vi "Process Records.vi"(4 "map from message info to indexes":T2, 5 "RT hardware channel data":T3[](array[typedef])=[{"channel #"=0, "channel handle"=0, "labels settings for RT"=[]}] {"labels settings for RT"."Label Timestamp Channel Data Reference" format="%.0x"; "labels settings for RT"."Word Initial Raw Value" format="%032.0f"; "labels settings for RT"."Label Disable/Trigger Channel Reference" format="%.0x"; "labels settings for RT"."parameter driver data"."Tx parameter refs" format="%.0x"; "labels settings for RT"."SDI" format="%02b"; "labels settings for RT"."label" format="%.0o"}, 6 "error in":errorcluster, 8 "map of message info to data word":T1(array[cluster]), 9 "parameter values in":dbl[](array[numeric])) -> (0 "error out":errorcluster, 3 "parameter values out":dbl[](array[numeric]))   [LabVIEW 2023, in "Ballard ARINC 429 Engine.lvlib" / "Custom Device.lvlib"]
uses:
  Custom Device.lvlib
  Shared/RT Hardware Channel Settings.ctl
  Shared/RT Label Settings.ctl
  Shared/Label.ctl
  Shared/RT Parameters.ctl
  Shared/Parameter Definition.ctl
  <vilib>/NI/NI VeriStand Encoding and Decoding/Encoding.ctl
  <vilib>/NI VeriStand/Custom Device API/Custom Device Item Ref.ctl
  Shared/Transfer Type.ctl
  <vilib>/NI VeriStand/Custom Device API/Data Reference.ctl
  Shared/Map of Identifiers to Indexes.ctl
  ece6b673-d70a-4abd-8fc5-cd5ecd079ce2.vi
  ece6b673-d70a-4abd-8fc5-cd5ecd079ce2.vi/1980749b-e417-4a21-943a-7c30016504b0.vi
  ece6b673-d70a-4abd-8fc5-cd5ecd079ce2.vi/1f3c3557-5c17-491c-9e18-ef0b55369bc3.vi
  ece6b673-d70a-4abd-8fc5-cd5ecd079ce2.vi/1980749b-e417-4a21-943a-7c30016504b0.vi/16a2565b-3c16-407b-a626-9da2a3da432e.vi
  ece6b673-d70a-4abd-8fc5-cd5ecd079ce2.vi/1f3c3557-5c17-491c-9e18-ef0b55369bc3.vi/0a001d06-2809-4638-8d0b-e017d2157007.vi
  ece6b673-d70a-4abd-8fc5-cd5ecd079ce2.vi/1f3c3557-5c17-491c-9e18-ef0b55369bc3.vi/e08d08e5-79bf-42ec-a5e5-c4db927cd1a5.vi
  <vilib>/NI/NI VeriStand Encoding and Decoding/Get Bits Per Digit from Base.vi
  <vilib>/NI VeriStand/Custom Device API/Custom Device API.lvlib
  <vilib>/NI/NI VeriStand Encoding and Decoding/Encoding and Decoding.lvlib
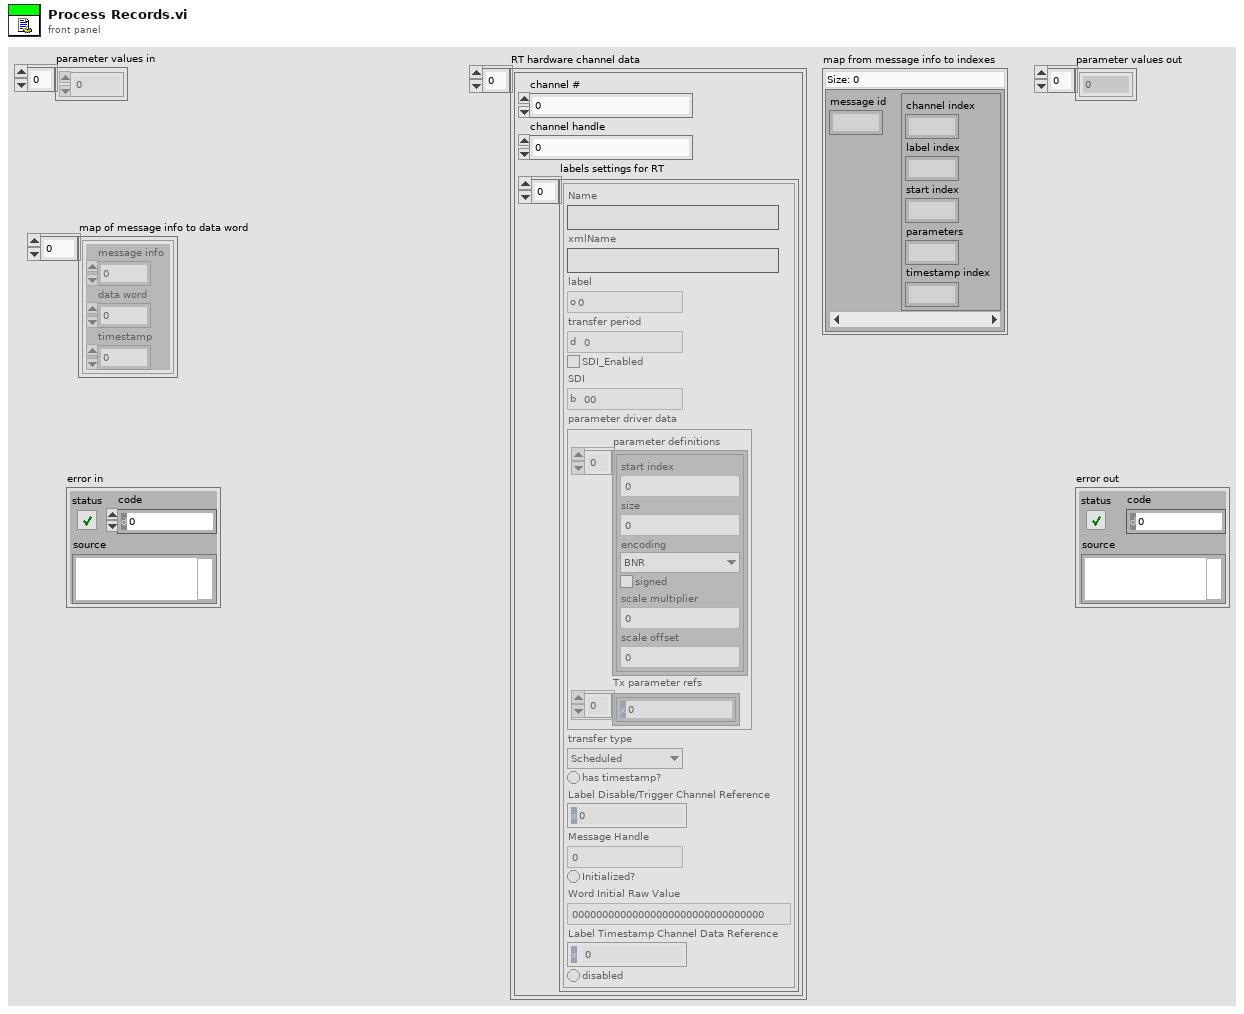
[diagram p1: front panel]
types:
  T1 = cluster{"message info":u32, "data word":u32, "timestamp":dbl}[]
  T2 = typedef "Map of Identifiers to Indexes.ctl" = map{u32, cluster{"channel index":i32, "label index":i32, "start index":i32, "parameters":i32, "timestamp index":i32}}
  T3 = typedef "RT Hardware Channel Settings.ctl" = cluster{"channel #":u16, "channel handle":u64, "labels settings for RT":T4[]}
  T4 = typedef "RT Label Settings.ctl" = cluster{"Name":string, "xmlName":string, "label":T5, "transfer period":u32, "SDI_Enabled":bool, "SDI":u8, "parameter driver data":T6, "transfer type":T10, "has timestamp?":bool, "Label Disable/Trigger Channel Reference":T9, "Message Handle":u64, "Initialized?":bool, "Word Initial Raw Value":u32, "Label Timestamp Channel Data Reference":T11, "disabled":bool}
  T5 = typedef "Label.ctl" = u8
  T6 = typedef "RT Parameters.ctl" = cluster{"parameter definitions":T7[], "Tx parameter refs":T9[]}
  T7 = typedef "Parameter Definition.ctl" = cluster{"start index":i32, "size":i32, "encoding":T8, "signed":bool, "scale multiplier":dbl, "scale offset":dbl}
  T8 = typedef "Encoding and Decoding.lvlib/Encoding.ctl" = enum16{"BNR", "BCD", "Discrete"}
  T9 = typedef "Custom Device API.lvlib/Custom Device Item Ref.ctl" = u64
  T10 = typedef "Transfer Type.ctl" = enum16{"Scheduled", "Acyclic", "Block", "Strobe"}
  T11 = typedef "Custom Device API.lvlib/Data Reference.ctl" = i32
  T12 = cluster{"channel index":i32, "label index":i32, "start index":i32, "parameters":i32, "timestamp":i32}
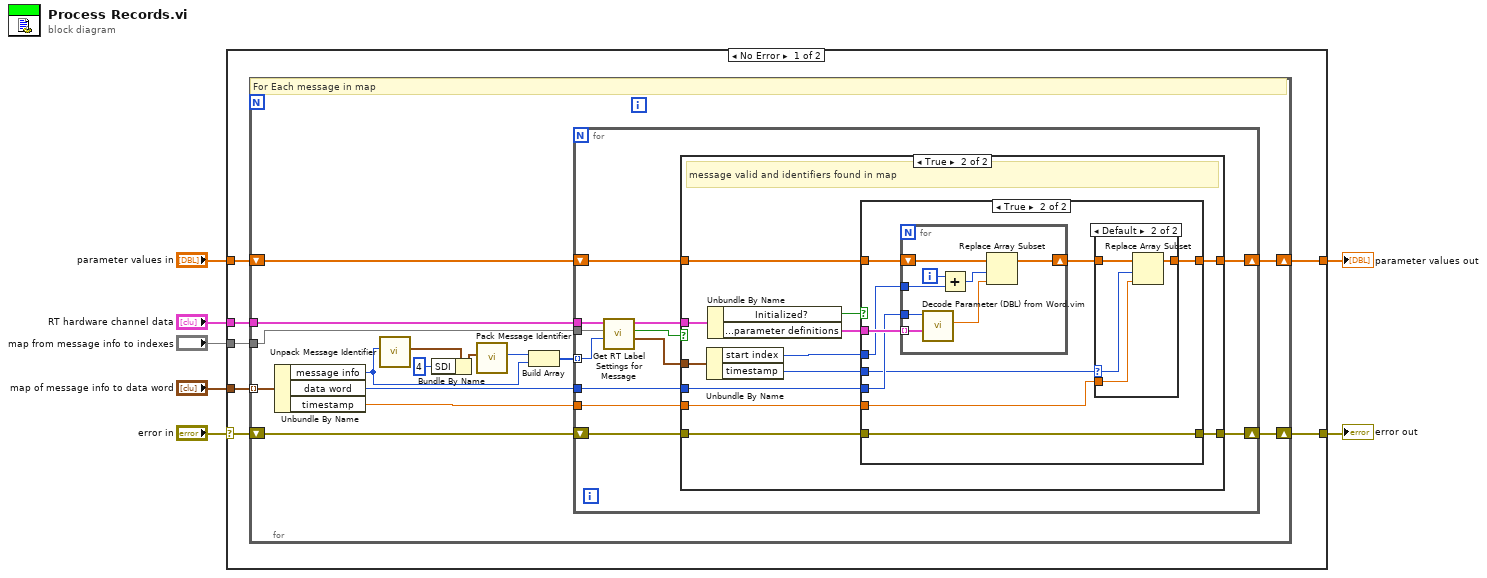
[diagram p0: block diagram]
diagram:
  n1 = case shown="No Error" "error in" {
    selector: "error in" -> [w12 w81]
    tunnel: "map of message info to data word" -> [w11 _]
    tunnel: [w14 w81] -> w7
    tunnel: "RT hardware channel data" -> [w13 _]
    tunnel: [w9 w80] -> w2
    tunnel: "parameter values in" -> [w10 w80]
    tunnel: "map from message info to indexes" -> [w8 _]
    frame No Error {
      n2 = for "Process each Record" {
        tunnel: w11 -> [w24] mode=indexing
        shift-right: [w29] -> w14
        shift-left: w12 -> [w28]
        tunnel: w13 -> [w27]
        shift-right: [w15] -> w9
        shift-left: w10 -> [w16]
        tunnel: w8 -> [w26]
        # "For Each message in map"
        n3 = Unbundle By Name(w24) -> ("message info"=w18:u32, "data word"=w25:u32, "timestamp"=w23:dbl)
        n4 = call "Unpack Message Identifier.vi"("packed message identifier"=w18) -> ("message identifiers"=w22:cluster{"Port":u8, "Label":u8, "SDI":u8})  [unwired: 10 in]
        n5 = Bundle By Name(cluster=w22, "SDI"=u8 4) -> (w20:cluster{"Port":u8, "Label":u8, "SDI":u8})
        n6 = call "Pack Message Identifier.vi"("message identifiers"=w20) -> ("packed message identifier"=w19:u32)  [unwired: 10 in]
        n7 = Build Array(w19, w18) -> (w17:u32[])
        n8 = for {
          tunnel: w27 -> [w38]
          tunnel: w26 -> [w33]
          tunnel: w25 -> [w35]
          tunnel: w23 -> [w34]
          shift-right: [w41] -> w29
          shift-left: w28 -> [w40]
          tunnel: w17 -> [w32] mode=indexing
          shift-right: [w31] -> w15
          shift-left: w16 -> [w39]
          n9 = call "Get RT Label Settings for Message.vi"("message identifier"=w32, "map"=w33, "RT hardware channel data"=w38) -> ("message indexes"=w36:T12, "valid and map exists"=w30:bool, "label settings for RT"=w37:T4)  [unwired: 6 in]
          n10 = case "Channel Found?" shown="True" w30 {
            tunnel: w40 -> [w43 w54]
            tunnel: [w43 w53] -> w41
            tunnel: w35 -> [_ w49]
            tunnel: [w42 w52] -> w31
            tunnel: w39 -> [w42 w50]
            tunnel: w37 -> [_ w48]
            tunnel: w36 -> [_ w47]
            tunnel: w34 -> [_ w45]
            frame False {
              # "message not valid or not found in map"
            }
            frame True {
              # "message valid and identifiers found in map"
              n11 = Unbundle By Name(w47) -> ("start index"=w46:i32, "timestamp"=w44:i32)
              n12 = Unbundle By Name(w48) -> ("Initialized?"=w51:bool, "parameter driver data.parameter definitions"=w55:T7[])
              n13 = case shown="True" w51 {
                tunnel: w55 -> [_ w65]
                tunnel: w49 -> [_ w64]
                tunnel: w54 -> [w57 w66]
                tunnel: [w57 w66] -> w53
                tunnel: [w56 w60] -> w52
                tunnel: w50 -> [w56 w63]
                tunnel: w46 -> [_ w62]
                tunnel: w45 -> [_ w58]
                tunnel: w44 -> [_ w61]
                frame False {
                  # "This case will be called if users has Labels present on the channel but didn't list them in XML file with \"monitor=false\" in the list.\n\nRecords returned by Read function will have labels (not filtered by HW)."
                }
                frame True {
                  n14 = for {
                    tunnel: w65 -> [w79] mode=indexing
                    tunnel: w64 -> [w73]
                    tunnel: w62 -> [w75]
                    shift-right: [w77] -> w59
                    shift-left: w63 -> [w78]
                    i -> [w76]
                    n15 = call "Decode Parameter (DBL) from Word.vim"("parameter definition"=w79, "32-bit word in"=w73) -> ("parameter value"=w72:dbl)  [unwired: 7 in, 2 out]
                    n16 = Add(x=w76, y=w75) -> (x+y=w74:i32)
                    n17 = Replace Array Subset(array=w78, new element=w72, index=w74) -> (w77:dbl[])
                  }
                  n18 = case shown="Default" w61 {
                    selector: w61 -> [_ w69]
                    tunnel: [w67 w70] -> w60
                    tunnel: w59 -> [w67 w71]
                    tunnel: w58 -> [_ w68]
                    frame ..-1 {
                    }
                    frame Default {
                      n19 = Replace Array Subset(array=w71, new element=w68, index=w69) -> (w70:dbl[])
                    }
                  }
                }
              }
            }
          }
        }
      }
    }
    frame Error {
    }
  }
  "error out" <- w7
  "parameter values out" <- w2
